vi "Clean Up Diagrams.vi"() -> ()   [LabVIEW 2020]
doc: "Dev helper: runs LabVIEW's Clean Up Diagram (BD.CleanUp, the options of Tools È Options È Block Diagram È Cleanup) on every VI listed in the items file (one path per line) and saves it for version (20.0 by default) in place, so a newer LabVIEW can run it: LabVIEW 2020's BD.CleanUp answers error 2. Close the VIs without saving afterwards. Returns the error code per item."
panel:
  out "error out":errorcluster
  out "codes":i32[](array[numeric])
  in  "version":string="20.0"
  in  "items file":path
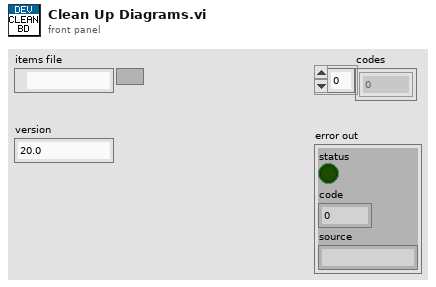
[diagram p1: front panel]
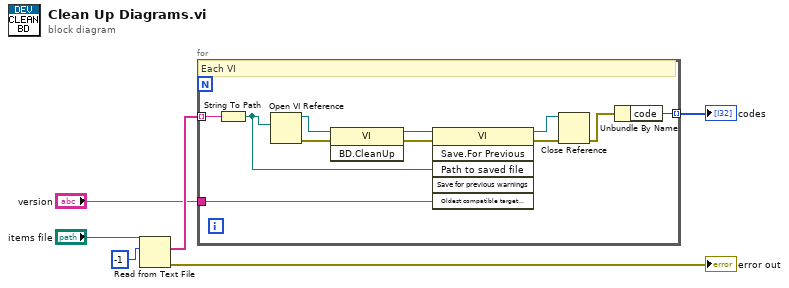
[diagram p0: block diagram]
diagram:
  n1 = Read from Text File(file (use dialog)="items file", count=-1) -> (text=w4:string[], error out=→"error out":errorcluster)  [unwired: 2 in, 2 out]
  n2 = for {
    tunnel: "version" -> [w8]
    tunnel: w4 -> [w7] mode=indexing
    tunnel: [w17] -> w6 mode=indexing
    # "Each VI"
    n3 = String To Path(string=w7) -> (path=w9:path)
    n4 = Open VI Reference(vi path=w9) -> (vi reference=w10:refnum<vi>, error out=w11:errorcluster)  [unwired: 5 in]
    n5 = invoke class="VI" method="BD.CleanUp"(reference=w10, error in=w11) -> (reference out=w12:refnum<vi>, error out=w13:errorcluster)  [unwired: 1 in, 1 out]
    n6 = invoke class="VI" method="Save.For Previous"(reference=w12, error in=w13, "Path to saved file"=w9, "Oldest compatible target version"=w8) -> (reference out=w14:refnum<vi>, error out=w15:errorcluster)  [unwired: 2 in, 4 out]
    n7 = Close Reference(reference=w14, error in (no error)=w15) -> (error out=w16:errorcluster)
    n8 = Unbundle By Name(w16) -> ("code"=w17:i32)
  }
  "codes" <- w6
